vi "command_current__28c2e5f573.vi"(8 "error in (no error)":errorcluster, 9 "relative seconds":dbl, 10 "output":dbl, 11 "IVI Refnum in":refnum<k15>) -> (0 "error out":errorcluster, 1 "Array":string[](array[string]), 2 "String":string, 3 "IVI Refnum out":refnum<k15>, 4 "Array 2":string[](array[string]), 5 "current measurements":dbl[](array[numeric]))   [LabVIEW 2023]
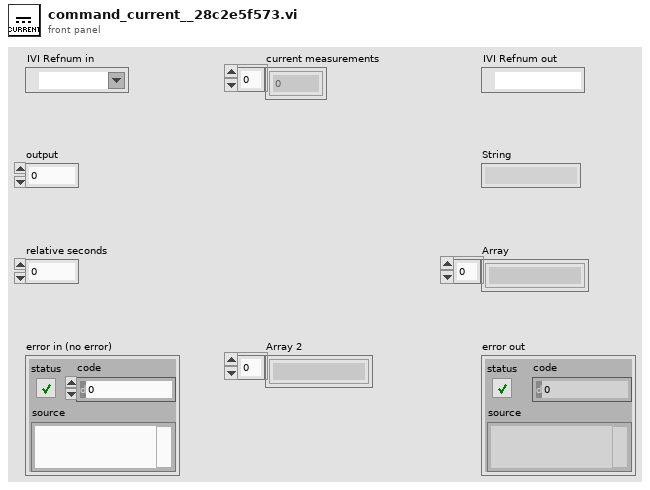
[diagram p1: front panel]
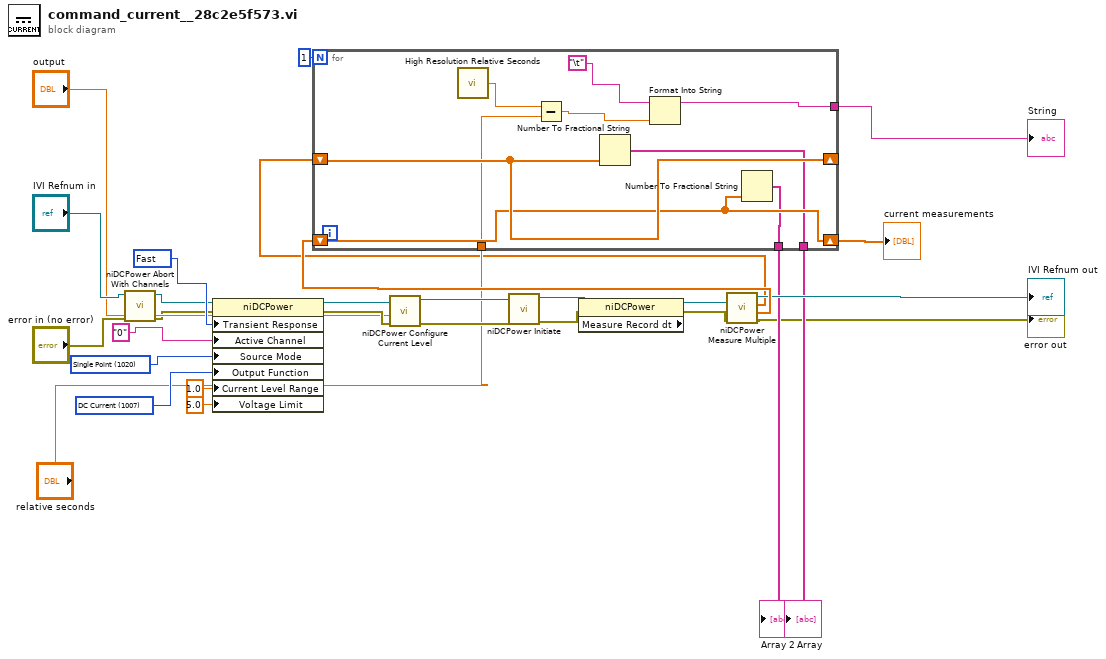
[diagram p0: block diagram]
diagram:
  w25 = 1007 items=["DC Voltage"=1006, "DC Current"=1007, "Pulse Voltage"=1049, "Pulse Current"=1050] ("Source:Output Function")
  w24 = 1020 items=["Single Point"=1020, "Sequence"=1021] ("Source:Source Mode")
  w4 = 1039 items=["Slow"=1041, "Normal"=1038, "Fast"=1039, "Custom"=1042] ("Source:Transient Response")
  n1 = call <instrlib>:"niDCPower Abort With Channels.vi"("error in (no error)"="error in (no error)", "instrument handle"="IVI Refnum in") -> ("error out"=w1:errorcluster, "instrument handle out"=w2:refnum<k15>)  [unwired: 8 in]
  n2 = property class="niDCPower"(reference=w2, error in=w1, "Transient Response"=w4, "Active Channel"="0", "Source Mode"=w24, "Output Function"=w25, "Current Level Range"=1.0 ("Source:DC Current:Current Level Range"), "Voltage Limit"=5.0 ("Source:DC Current:Voltage Limit")) -> (reference out=w8:refnum<k15>, error out=w9:errorcluster)
  n3 = call <instrlib>:"niDCPower Configure Current Level.vi"("error in (no error)"=w9, "current level"="output", "instrument handle"=w8) -> ("error out"=w23:errorcluster, "instrument handle out"=w22:refnum<k15>)  [unwired: 7 in]
  n4 = call <instrlib>:"niDCPower Initiate.vi"("error in (no error)"=w23, "instrument handle"=w22) -> ("error out"=w11:errorcluster, "instrument handle out"=w10:refnum<k15>)  [unwired: 2 in, 6 out]
  n5 = property class="niDCPower" props=["Measure Record dt"](reference=w10, error in=w11) -> (reference out=w20:refnum<k15>, error out=w21:errorcluster)  [unwired: 1 out]
  n6 = call <instrlib>:"niDCPower Measure Multiple.vi"("error in (no error)"=w21, "instrument handle"=w20) -> ("error out"=→"error out":errorcluster, "current measurements"=w28:dbl[], "voltage measurements"=w14:dbl[], "instrument handle out"=→"IVI Refnum out":refnum<k15>)  [unwired: 6 in]
  n7 = for {
    N: 1 -> [_]
    tunnel: [w37] -> w13
    shift-right: [w36] -> _
    shift-left: w14 -> [w36]
    shift-right: [w35] -> w29
    shift-left: w28 -> [w35]
    tunnel: [w34] -> w16
    tunnel: "relative seconds" -> [w32]
    tunnel: [w30] -> w18
    n8 = call <vilib>:"High Resolution Relative Seconds.vi"() -> ("relative seconds"=w31:dbl)
    n9 = Subtract(x=w31, y=w32) -> (x-y=w38:dbl)
    n10 = Number To Fractional String(number=w36) -> (F-format string=w30:string[])  [unwired: 3 in]
    n11 = Format Into String(initial string="\t", w38) -> (resulting string=w37:string)  [unwired: 2 in, 1 out]
    n12 = Number To Fractional String(number=w35) -> (F-format string=w34:string[])  [unwired: 3 in]
  }
  "current measurements" <- w29
  "Array" <- w18
  "Array 2" <- w16
  "String" <- w13
